vi "Arithmetic-Calculator.vi"() -> ()   [LabVIEW 2026]
panel:
  out "error in (no error)":errorcluster
  out "RESULT":dbl
  in  "CALCULATE":bool
  in  "MODE":enum16{"SUB", "DIV", "MUL", "ADD"}(ring)
  in  "value 2":dbl
  in  "value":dbl
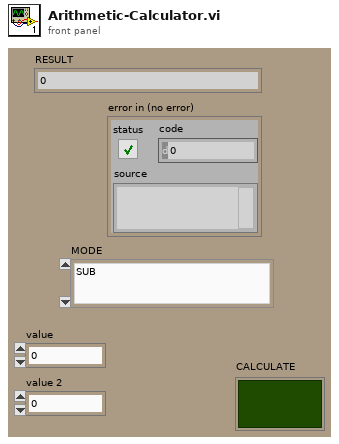
[diagram p1: front panel]
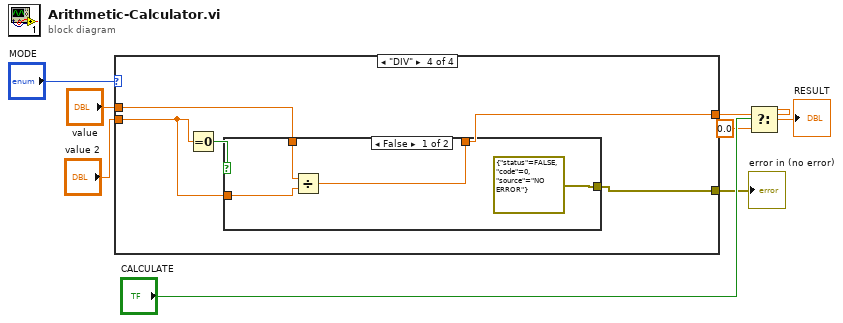
[diagram p0: block diagram]
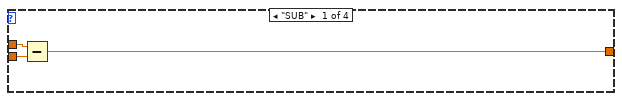
[diagram p2: hidden frame]
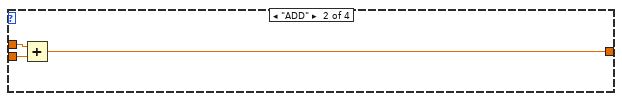
[diagram p3: hidden frame]
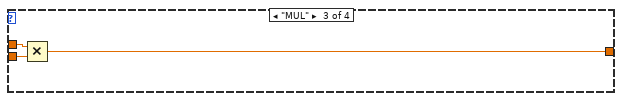
[diagram p4: hidden frame]
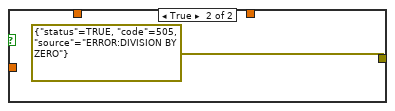
[diagram p5: hidden frame]
diagram:
  n1 = case shown="\"DIV\"" "MODE" {
    tunnel: "value" -> [w11 w14 w17 w20]
    tunnel: "value 2" -> [w10 w13 w16 w21]
    tunnel: [w9 w12 w15 w19] -> w5
    tunnel: [_ _ _ w18] -> w1
    frame "SUB" {
      n2 = Subtract(x=w11, y=w10) -> (x-y=w9:dbl)
    }
    frame "ADD" {
      n3 = Add(x=w14, y=w13) -> (x+y=w12:dbl)
    }
    frame "MUL" {
      n4 = Multiply(x=w17, y=w16) -> (x*y=w15:dbl)
    }
    frame "DIV" {
      n5 = Equal To 0?(x=w21) -> (x = 0?=w22:bool)
      n6 = case shown="False" w22 {
        tunnel: w21 -> [w24 _]
        tunnel: w20 -> [w26 _]
        tunnel: [w25 _] -> w19
        tunnel: [errorcluster {"status"=FALSE, "code"=0, "source"="NO ERROR"} ("error constant") errorcluster {"status"=TRUE, "code"=505, "source"="ERROR:DIVISION BY ZERO"} ("error constant")] -> w18
        frame False {
          n7 = Divide(x=w26, y=w24) -> (x/y=w25:dbl)
        }
        frame True {
        }
      }
    }
  }
  "error in (no error)" <- w1
  n8 = Select(t=w5, s="CALCULATE", f=0.0) -> (s? t:f=→"RESULT":dbl)
